vi "LM35 Interface with Arduino.vi"() -> ()   [LabVIEW 2014]
uses:
  <vilib>/LabVIEW Interface for Arduino/Type Defs/Board Type.ctl
  <vilib>/LabVIEW Interface for Arduino/Type Defs/Connection Type.ctl
  <vilib>/LabVIEW Interface for Arduino/LabVIEW Interface for Arduino.lvlib
panel:
  in  "Very Hot Led Pin":u8
  in  "Hot Led Pin":u8
  in  "Moderate Led Pin":u8
  in  "Cool Led Pin":u8
  in  "Fan Pin":u8
  in  "Connection Type (USB/Serial)":T1
  in  "Board Type (Uno)":T2
  in  "VISA resource":refnum<visa-resource-name>
  in  "Temp Read Pin":u8
  out "Meter":dbl(knob) scale=-1.0..1.5
  out "Sensor Voltage":dbl
  out "Thermometer":dbl(slide) scale=0.0..100.0
  out "Temperature C":dbl
  in  "stop":bool
  out "Cool":bool
  out "Moderate":bool
  out "Hot":bool
  out "Very Hot":bool
  # "LabVIEW interface with Arduino for Temperature Measurement Using LM-35"
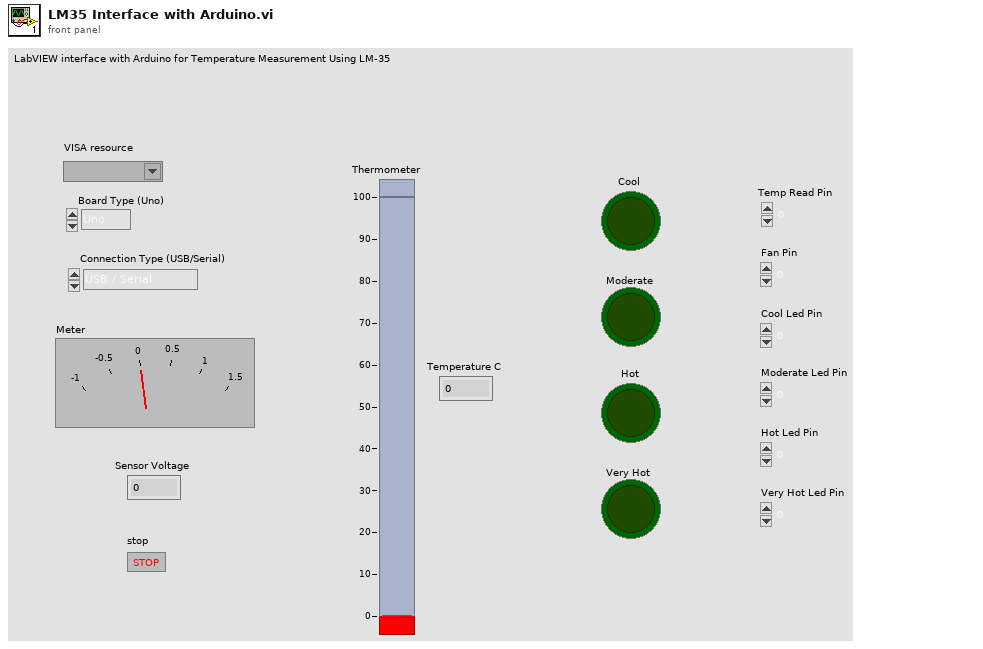
[diagram p1: front panel]
types:
  T1 = typedef "LabVIEW Interface for Arduino.lvlib/Connection Type.ctl" = enum8{"USB / Serial", "XBEE", "BlueSmirf (Bluetooth)"}
  T2 = typedef "LabVIEW Interface for Arduino.lvlib/Board Type.ctl" = enum16{"Uno", "Dimuelanove w/Atmega 328", "Mega 2560"}
  T3 = typedef "LabVIEW Interface for Arduino.lvlib/Arduino Resource.ctl" = cluster{"VISA resource":refnum<visa-resource-name>, "Board Type":T2, "Connection Type":enum8{"USB / Serial"}, "Bytes Per Packet (15)":u8}
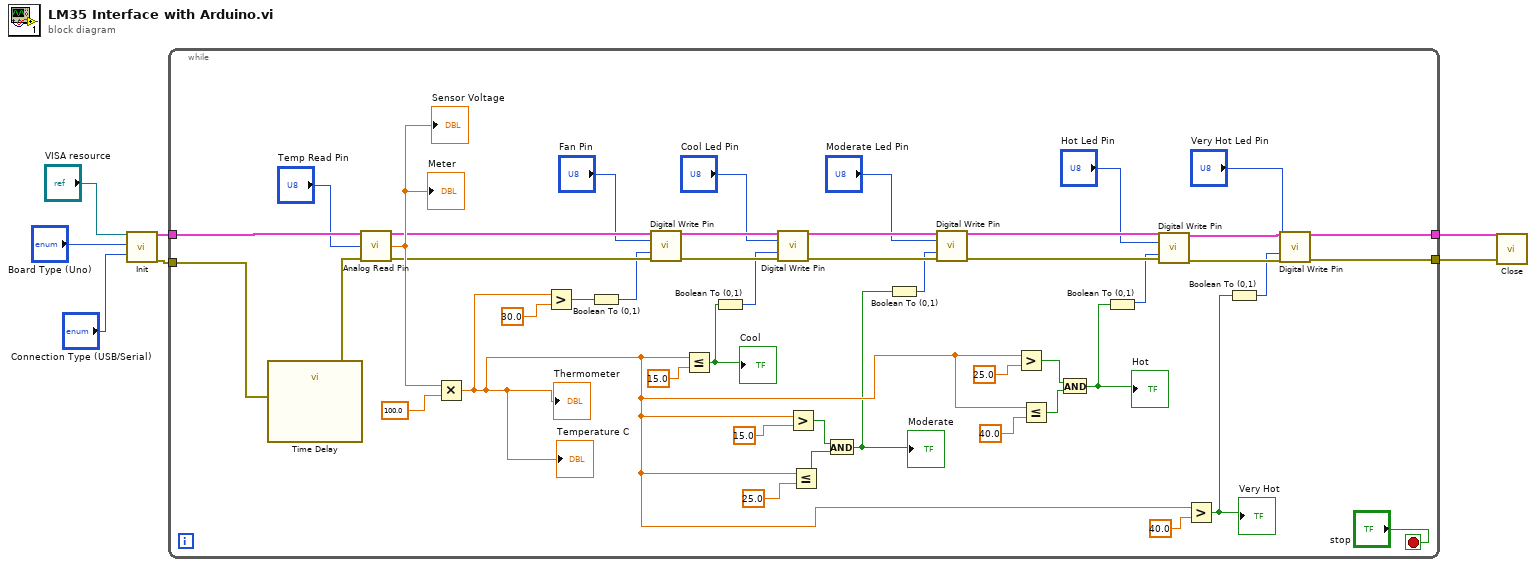
[diagram p0: block diagram]
diagram:
  n1 = call <vilib>:"Init.vi"("VISA resource"="VISA resource", "Board Type (Uno)"="Board Type (Uno)", "Connection Type (USB/Serial)"="Connection Type (USB/Serial)") -> ("Arduino Resource"=w7:T3, "error out"=w6:errorcluster)  [unwired: 15 in]
  n2 = while {
    tunnel: w7 -> [w53]
    tunnel: w6 -> [w48]
    tunnel: [w12] -> w2
    tunnel: [w11] -> w1
    stop <- "stop" stop-if-true
    n3 = call "Time Delay"("error in (no error)"=w48) -> ("error out"=w49:errorcluster)  [unwired: 10 in]
    n4 = call <vilib>:"Analog Read Pin.vi"("Arduino Resource"=w53, "Analog Input Pin (0)"="Temp Read Pin", "error in"=w49) -> ("Arduino Resource"=w35:T3, "Voltage"=w37:dbl, "error out"=w34:errorcluster)  [unwired: 10 in]
    "Meter" <- w37
    "Sensor Voltage" <- w37
    n5 = Multiply(x=w37, y=100.0) -> (x*y=w32:dbl)
    "Thermometer" <- w32
    "Temperature C" <- w32
    n6 = Greater?(x=w32, y=30.0) -> (0:w31:bool)
    n7 = Boolean To (0,1)(Boolean=w31) -> (0, 1=w33:i16)
    n8 = call <vilib>:"Digital Write Pin.vi"("Arduino Resource"=w35, "Digital I/O Pin (0)"="Fan Pin", "Value (0)"=w33, "error in"=w34) -> ("Arduino Resource"=w30:T3, "error out"=w29:errorcluster)  [unwired: 10 in]
    n9 = Less Or Equal?(x=w32, y=15.0) -> (x <= y?=w25:bool)
    "Cool" <- w25
    n10 = Boolean To (0,1)(Boolean=w25) -> (0, 1=w26:i16)
    n11 = call <vilib>:"Digital Write Pin.vi"("Arduino Resource"=w30, "Digital I/O Pin (0)"="Cool Led Pin", "Value (0)"=w26, "error in"=w29) -> ("Arduino Resource"=w24:T3, "error out"=w23:errorcluster)  [unwired: 10 in]
    n12 = Greater?(x=w32, y=15.0) -> (0:w41:bool)
    n13 = Less Or Equal?(x=w32, y=25.0) -> (x <= y?=w40:bool)
    n14 = And(x=w41, y=w40) -> (x .and. y?=w22:bool)
    "Moderate" <- w22
    n15 = Boolean To (0,1)(Boolean=w22) -> (0, 1=w21:i16)
    n16 = call <vilib>:"Digital Write Pin.vi"("Arduino Resource"=w24, "Digital I/O Pin (0)"="Moderate Led Pin", "Value (0)"=w21, "error in"=w23) -> ("Arduino Resource"=w19:T3, "error out"=w18:errorcluster)  [unwired: 10 in]
    n17 = Greater?(x=w32, y=25.0) -> (0:w38:bool)
    n18 = Less Or Equal?(x=w32, y=40.0) -> (x <= y?=w39:bool)
    n19 = And(x=w38, y=w39) -> (x .and. y?=w16:bool)
    "Hot" <- w16
    n20 = Boolean To (0,1)(Boolean=w16) -> (0, 1=w17:i16)
    n21 = call <vilib>:"Digital Write Pin.vi"("Arduino Resource"=w19, "Digital I/O Pin (0)"="Hot Led Pin", "Value (0)"=w17, "error in"=w18) -> ("Arduino Resource"=w14:T3, "error out"=w13:errorcluster)  [unwired: 10 in]
    n22 = Greater?(x=w32, y=40.0) -> (0:w8:bool)
    "Very Hot" <- w8
    n23 = Boolean To (0,1)(Boolean=w8) -> (0, 1=w9:i16)
    n24 = call <vilib>:"Digital Write Pin.vi"("Arduino Resource"=w14, "Digital I/O Pin (0)"="Very Hot Led Pin", "Value (0)"=w9, "error in"=w13) -> ("Arduino Resource"=w12:T3, "error out"=w11:errorcluster)  [unwired: 10 in]
  }
  n25 = call <vilib>:"Close.vi"("Arduino Resource"=w2, "error in"=w1) -> ()  [unwired: 13 in, 1 out]
